vi "VIH Utility - FILE - Relative Path from Absolute Path.vi"(7 "base path (empty: dir of Top VI)":path, 8 "error in":errorcluster, 11 "Path":path) -> (0 "error out":errorcluster, 3 "Rel Path out":path, 5 "Common Path out":path)   [LabVIEW 2014]
doc: "::: VI Helpeks :::\nCopyright (c) 2000-2026 Konstantin Shifershteyn. All rights reserved."
panel:
  # "VI Helpeks\nCopyright (c) 2012-2026 Konstantin Shifershteyn"
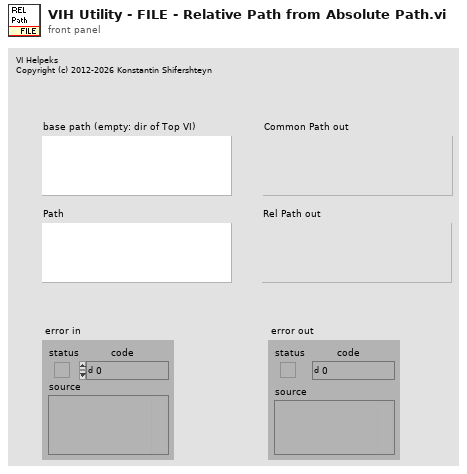
[diagram p1: front panel]
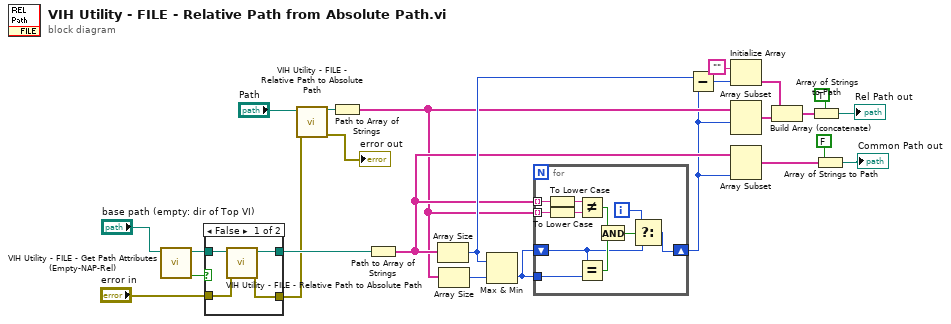
[diagram p0: block diagram]
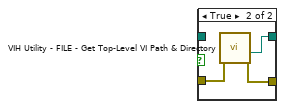
[diagram p2: hidden frame]
diagram:
  n1 = call "VIH Utility - FILE - Get Path Attributes (Empty-NAP-Rel).vi"("Path"="base path (empty: dir of Top VI)") -> ("Not A Path or Empty path"=w18:bool, "dup Path"=w19:path)  [unwired: 9 out]
  n2 = case shown="False" w18 {
    tunnel: [w27 w30] -> w24
    tunnel: w19 -> [w26 _]
    tunnel: "error in" -> [w28 w32]
    tunnel: [w29 w31] -> w21
    frame False {
      n3 = call "VIH Utility - FILE - Relative Path to Absolute Path.vi"("error in"=w28, "Path"=w26) -> ("error out"=w29:errorcluster, "Path out"=w27:path)  [unwired: 1 in, 7 out]
    }
    frame True {
      n4 = call "VIH Utility - FILE - Get Top-Level VI Path & Directory.vi"("error in"=w32) -> ("error out"=w31:errorcluster, "VI Directory out of .LLB"=w30:path)  [unwired: 9 out]
    }
  }
  n5 = call "VIH Utility - FILE - Relative Path to Absolute Path.vi"("error in"=w21, "Path"="Path") -> ("error out"=→"error out":errorcluster, "Path out"=w23:path)  [unwired: 1 in, 7 out]
  n6 = Path to Array of Strings(0:w23) -> (2:w5:string[])  [unwired: 1 out]
  n7 = Path to Array of Strings(0:w24) -> (2:w6:string[])  [unwired: 1 out]
  n8 = Array Size(array=w6) -> (size(s)=w9:i32)
  n9 = Array Size(array=w5) -> (size(s)=w8:i32)
  n10 = Max & Min(x=w9, y=w8) -> (min(x,y)=w7:i32)  [unwired: 1 out]
  n11 = for {
    tunnel: w6 -> [w43] mode=indexing
    tunnel: w5 -> [w42] mode=indexing
    shift-right: [w35] -> w2
    shift-left: w7 -> [w36]
    tunnel: w7 -> [w41]
    i -> [w37]
    n12 = To Lower Case(string=w43) -> (all lower case string=w34:string)
    n13 = To Lower Case(string=w42) -> (all lower case string=w33:string)
    n14 = Not Equal?(x=w34, y=w33) -> (x != y?=w39:bool)
    n15 = Equal?(x=w36, y=w41) -> (x = y?=w40:bool)
    n16 = And(x=w39, y=w40) -> (x .and. y?=w38:bool)
    n17 = Select(t=w37, s=w38, f=w36) -> (s? t:f=w35:i32)
  }
  n18 = Subtract(x=w9, y=w2) -> (x-y=w14:i32)
  n19 = Initialize Array("", w14) -> (w13:string[])
  n20 = Array Subset(array=w5, index=w2) -> (w12:string[])  [unwired: 1 in]
  n21 = Array Subset(array=w6, length=w2) -> (w15:string[])  [unwired: 1 in]
  n22 = Build Array (concatenate)(w13, w12) -> (w11:string[])
  n23 = Array of Strings to Path(0:w11, 1:TRUE ("relative")) -> (2:→"Rel Path out":path)
  n24 = Array of Strings to Path(0:w15, 1:FALSE ("relative")) -> (2:→"Common Path out":path)
